vi "ASD Time point for Graph VI.vi"(11 "Region Raw data":dbl[](array[numeric])) -> (3 "Time for Graph":i32[](array[numeric]))   [LabVIEW 2018]
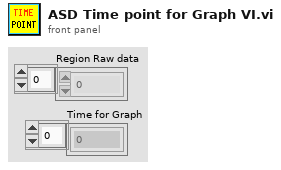
[diagram p1: front panel]
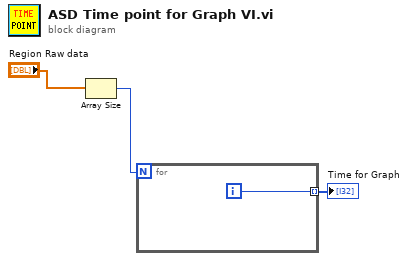
[diagram p0: block diagram]
diagram:
  n1 = Array Size(array="Region Raw data") -> (size(s)=w2:i32)
  n2 = for {
    N: w2 -> [_]
    tunnel: [w4] -> w1 mode=indexing
    i -> [w4]
  }
  "Time for Graph" <- w1
